vi "refresh table.vi"(5 "more filters":T1, 7 "Filter":string, 8 "error in":errorcluster, 9 "Table":refnum<vi>, 10 "taglist":refnum<data-value>, 11 "engine configuration in":refnum<class "engine configuration.lvclass">) -> (0 "error out":errorcluster)   [LabVIEW 2013, in "PL Framework Configuration Tool.lvlib" / "EngineTags.lvclass"]
uses:
  EngineTags.lvclass
  <vilib>/NI/Module Execution Interface/Engine Configuration/engine configuration.lvclass
  additional filter.ctl
  <vilib>/NI/Module Execution Interface/Engine Configuration/engine configuration.lvclass/engine configuration.ctl
  <vilib>/NI/Tag Bus/tag/tag descriptor.lvclass/tag descriptor.ctl
  EngineTags.lvclass/EngineTags.ctl
  <vilib>/NI/Tag Bus/tag/read tag name.vi
  <vilib>/NI/Tag Bus/tag/read data type.vi
  <vilib>/NI/Tag Bus/tag/read metadata.vi
  Read Sorting Enabled.vi
  Read Sorting Column.vi
  <vilib>/NI/Tag Bus/tag/tag descriptor.lvclass
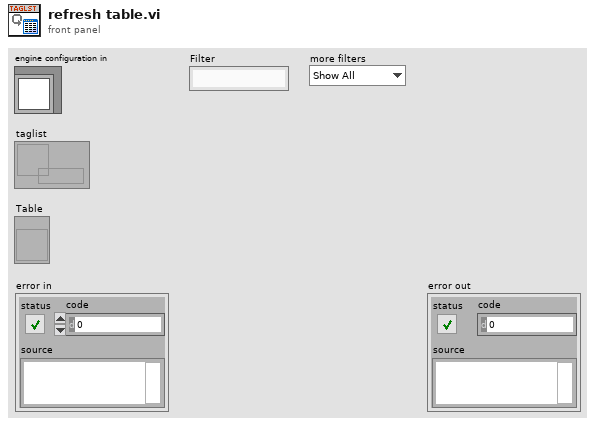
[diagram p1: front panel]
types:
  T1 = typedef "PL Framework Configuration Tool.lvlib/EngineTags.lvclass/additional filter.ctl" = enum16{"Show All", "Show Unmapped", "Show Tags with no Writer", "Show Tags with no Readers"}
  T2 = typedef "engine configuration.lvclass/unique channel identifier.ctl" = cluster{"channel":string, "module ID":string}
  T3 = typedef "tag bus.lvlib/tag descriptor.lvclass/Data Type.ctl" = enum16{"Double", "Single", "I64", "I32", "I16", "I8", "U64", "U32", "U16", "U8", "Boolean", "String", "Array of Double", "Array of Single", "Array of I64", "Array of I32", "Array of I16", "Array of I8", "Array of U64", "Array of U32", "Array of U16", "Array of U8", "Array of Boolean", "Array of String"}
  T4 = typedef "PL Framework Configuration Tool.lvlib/EngineTags.lvclass/sorting type.ctl" = enum16{"none", "asc", "desc"}
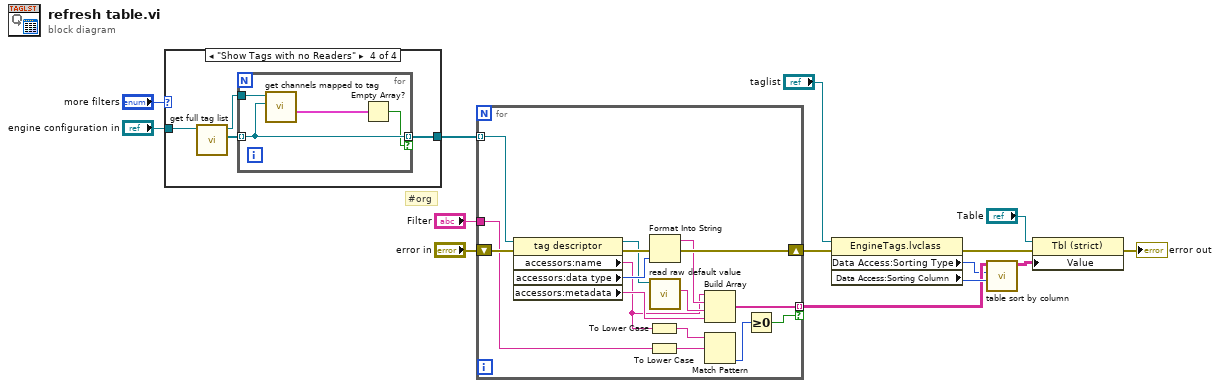
[diagram p0: block diagram]
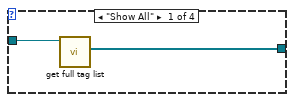
[diagram p2: hidden frame]
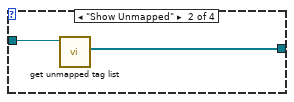
[diagram p3: hidden frame]
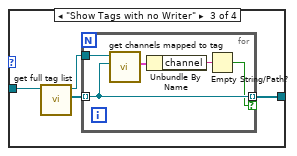
[diagram p4: hidden frame]
diagram:
  # "#org"
  n1 = case shown="\"Show Tags with no Readers\"" "more filters" {
    tunnel: [w16 w17 w19 w28] -> w7
    tunnel: "engine configuration in" -> [w15 w18 w21 w30]
    frame "Show All" {
      n2 = call <vilib>:"get full tag list.vi"("engine configuration in"=w15) -> ("tag list"=w16:refnum<class "tag descriptor.lvclass">[])  [unwired: 9 in, 1 out]
    }
    frame "Show Unmapped" {
      n3 = call <vilib>:"get unmapped tag list.vi"("engine configuration in"=w18) -> ("tag list"=w17:refnum<class "tag descriptor.lvclass">[])  [unwired: 9 in, 1 out]
    }
    frame "Show Tags with no Writer" {
      n4 = call <vilib>:"get full tag list.vi"("engine configuration in"=w21) -> ("tag list"=w22:refnum<class "tag descriptor.lvclass">[], "engine configuration out"=w20:refnum<class "engine configuration.lvclass">)  [unwired: 9 in]
      n5 = for {
        tunnel: w22 -> [w26] mode=indexing
        tunnel: w20 -> [w27]
        tunnel: [w26] -> w19 mode=indexing if=w23
        n6 = call <vilib>:"get channels mapped to tag.vi"("tag"=w26, "engine configuration in"=w27) -> ("writer"=w25:T2)  [unwired: 6 in, 3 out]
        n7 = Unbundle By Name(w25) -> ("channel"=w24:string)
        n8 = Empty String/Path?(string/path=w24) -> (empty?=w23:bool)
      }
    }
    frame "Show Tags with no Readers" {
      n9 = call <vilib>:"get full tag list.vi"("engine configuration in"=w30) -> ("tag list"=w31:refnum<class "tag descriptor.lvclass">[], "engine configuration out"=w29:refnum<class "engine configuration.lvclass">)  [unwired: 9 in]
      n10 = for {
        tunnel: w31 -> [w34] mode=indexing
        tunnel: w29 -> [w35]
        tunnel: [w34] -> w28 mode=indexing if=w33
        n11 = call <vilib>:"get channels mapped to tag.vi"("tag"=w34, "engine configuration in"=w35) -> ("readers"=w32:T2[])  [unwired: 6 in, 3 out]
        n12 = Empty Array?(array=w32) -> (empty?=w33:bool)
      }
    }
  }
  n13 = for {
    shift-right: [w48] -> w5
    shift-left: "error in" -> [w51]
    tunnel: w7 -> [w50] mode=indexing
    tunnel: [w42] -> w9 mode=indexing if=w40
    tunnel: "Filter" -> [w36]
    n14 = property class="tag descriptor"(reference=w50, error in=w51) -> (reference out=w46:refnum<class "tag descriptor.lvclass">, error out=w49:errorcluster, "accessors:name"=w38:string, "accessors:data type"=w47:T3, "accessors:metadata"=w44:string)
    n15 = To Lower Case(string=w38) -> (all lower case string=w39:string)
    n16 = To Lower Case(string=w36) -> (all lower case string=w37:string)
    n17 = Format Into String(error in=w49, w47) -> (resulting string=w45:string, error out=w48:errorcluster)  [unwired: 2 in]
    n18 = call <vilib>:"read raw default value.vi"("system tag in"=w46) -> ("raw default"=w43:string)  [unwired: 8 in, 2 out]
    n19 = Build Array(w38, w45, w43, w44) -> (w42:string[])
    n20 = Match Pattern(string=w39, regular expression=w37) -> (offset past match=w41:i32)  [unwired: 1 in, 3 out]
    n21 = Greater Or Equal To 0?(x=w41) -> (x >= 0?=w40:bool)
  }
  n22 = property class="EngineTags.lvclass"(reference="taglist", error in=w5) -> (error out=w4:errorcluster, "Data Access:Sorting Type"=w3:T4, "Data Access:Sorting Column"=w11:i32)  [unwired: 1 out]
  n23 = call "table sort by column.vi"("Column to sort"=w11, "Sorting Type"=w3, "Array"=w9) -> ("sorted array"=w14:string[][])  [unwired: 8 in]
  n24 = property on="Property Node" class="Tbl (strict)"(reference="Table", error in=w4, "Value"=w14) -> (error out=→"error out":errorcluster)  [unwired: 1 out]
